vi "Modbus Slave.vi"() -> ()   [LabVIEW 2021]
uses:
  <vilib>/NI/Modbus Library/API/Wrapper/Create TCP Slave.vi
  <vilib>/NI/Modbus Library/API/Slave/Modbus Slave.lvclass
  <vilib>/NI/Modbus Library/API/Wrapper/API Main.lvlib
panel:
  in  "Thermometer":u16(slide) scale=0.0..100.0
  out "error out 2":errorcluster
  in  "Elevator Control":u16(slide) scale=0.0..256.0
  in  "stop":bool
  in  "port (502)":u16=502
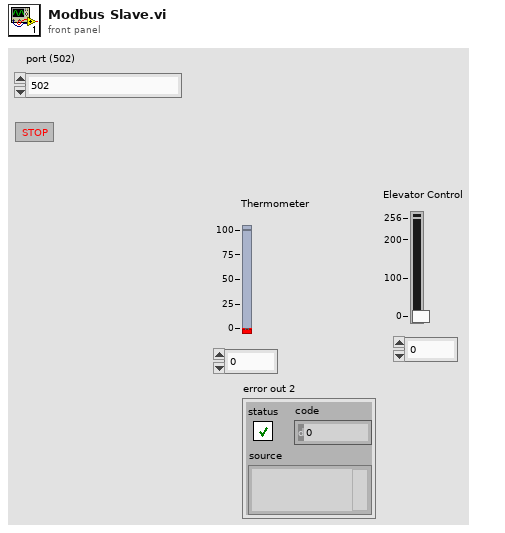
[diagram p1: front panel]
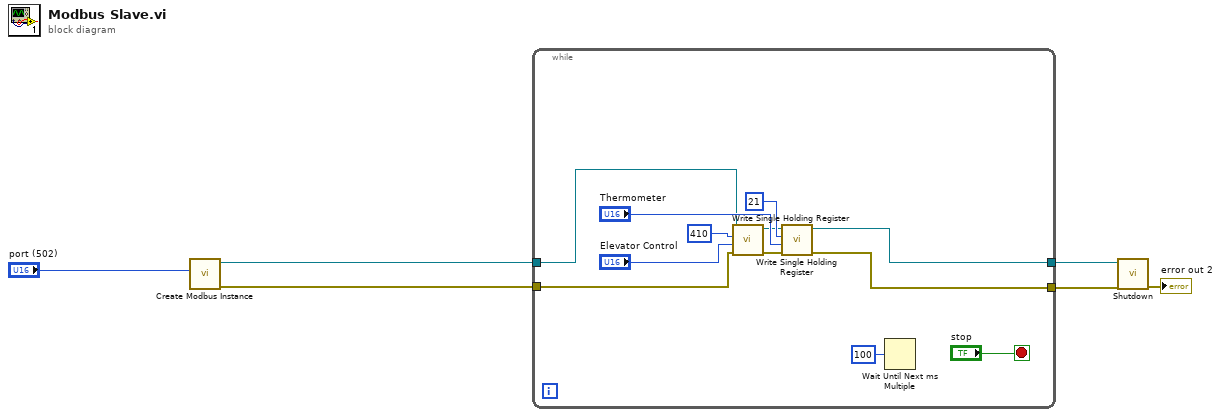
[diagram p0: block diagram]
diagram:
  n1 = call-poly <vilib>:"Create Modbus Instance.vi"("port (502)"="port (502)") -> ("error out"=w4:errorcluster, "TCP slave instance"=w5:refnum<class "Modbus Slave.lvclass">)  [unwired: 9 in]
  n2 = while {
    tunnel: w5 -> [w11]
    tunnel: w4 -> [w16]
    tunnel: [w9] -> w2
    tunnel: [w7] -> w3
    stop <- "stop" stop-if-true
    n3 = call-dynamic "Write Single Holding Register.vi"("error in"=w16, "register to write"="Elevator Control", "address"=u16 410, "Modbus slave in"=w11) -> ("error out"=w10:errorcluster, "Modbus slave out"=w8:refnum<class "Modbus Slave.lvclass">)  [unwired: 6 in]
    n4 = call-dynamic "Write Single Holding Register.vi"("error in"=w10, "register to write"="Thermometer", "address"=u16 21, "Modbus slave in"=w8) -> ("error out"=w9:errorcluster, "Modbus slave out"=w7:refnum<class "Modbus Slave.lvclass">)  [unwired: 6 in]
    n5 = Wait Until Next ms Multiple(millisecond multiple=u32 100) -> ()  [unwired: 1 out]
  }
  n6 = call-dynamic "Shutdown.vi"("error in"=w2, "Modbus slave in"=w3) -> ("error out"=→"error out 2":errorcluster)  [unwired: 9 in]
